vi "Y-Axis_step.vi"(9 "Up?":bool, 10 "Y Motor":refnum<k7>, 11 "Number of Y steps":dbl=1.0) -> (1 "Y indecator":i32)   [LabVIEW 2024]
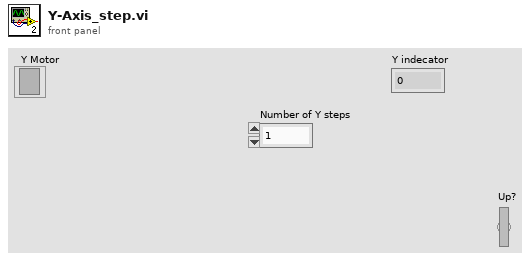
[diagram p1: front panel]
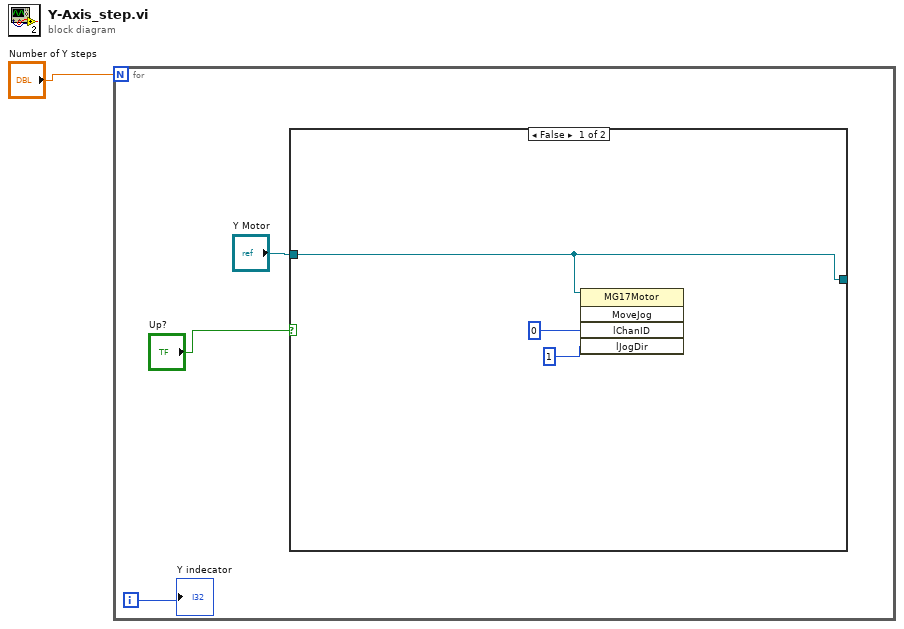
[diagram p0: block diagram]
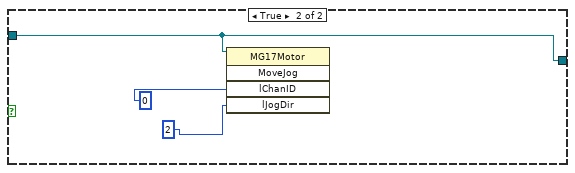
[diagram p2: hidden frame]
diagram:
  n1 = for {
    N: "Number of Y steps" -> [_]
    i -> [w2]
    n2 = case shown="False" "Up?" {
      tunnel: "Y Motor" -> [w5 w8]
      tunnel: [w5 w8] -> _
      frame False {
        n3 = invoke class="MG17Motor" method="MoveJog"(reference=w5, "lChanID"=0, "lJogDir"=1) -> ()  [unwired: 2 in, 5 out]
      }
      frame True {
        n4 = invoke class="MG17Motor" method="MoveJog"(reference=w8, "lChanID"=0, "lJogDir"=2) -> ()  [unwired: 2 in, 5 out]
      }
    }
    "Y indecator" <- w2
  }
